vi "SetRunOptions.vi"(7 "Options":T1={"exclude instances?"=FALSE, "exclude external? (T)"=TRUE, "separate tests?"=FALSE, "top level results only?"=FALSE, "Export options"={"Export rules"=FALSE, "Export dependencies"=FALSE, "Export invalid dependencies"=FALSE, "Export concessions"=FALSE, "Export undeclared"=FALSE}, "Filter options"={"Source filter"=refnum, "Target filter"=refnum, "AND Condition?"=FALSE}}, 8 "error in (no error)":errorcluster, 10 "Root path":path, 11 "CDependencyInspection in":refnum<class "CDependencyInspection.lvclass">) -> (0 "error out":errorcluster, 3 "CDependencyInspection out":refnum<class "CDependencyInspection.lvclass">)   [LabVIEW 2020, in "DependencyInspection.lvlib" / "CDependencyInspection.lvclass"]
uses:
  CDependencyInspection.lvclass
  Options.ctl
  Options_Export.ctl
  Options_Filter.ctl
  CDependencyInspection.lvclass/CDependencyInspection.ctl
  CItemMatch/CItemMatch.lvclass
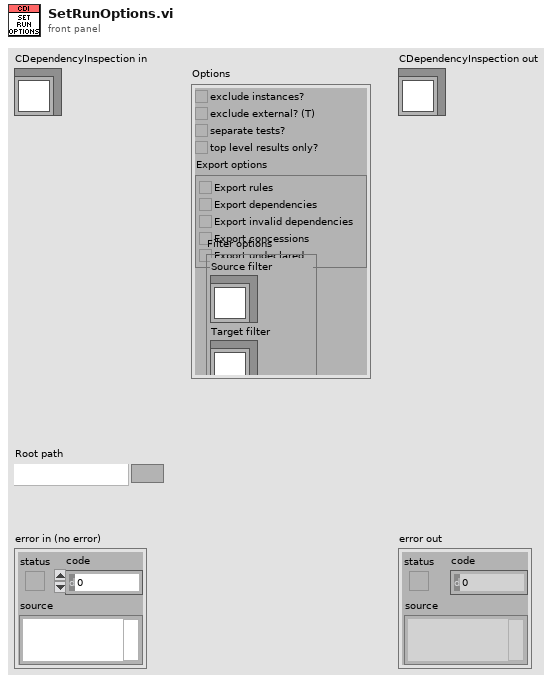
[diagram p1: front panel]
types:
  T1 = typedef "DependencyInspection.lvlib/CDependencyInspection.lvclass/Options.ctl" = cluster{"exclude instances?":bool, "exclude external? (T)":bool, "separate tests?":bool, "top level results only?":bool, "Export options":T2, "Filter options":T3}
  T2 = typedef "DependencyInspection.lvlib/CDependencyInspection.lvclass/Options_Export.ctl" = cluster{"Export rules":bool, "Export dependencies":bool, "Export invalid dependencies":bool, "Export concessions":bool, "Export undeclared":bool}
  T3 = typedef "DependencyInspection.lvlib/CDependencyInspection.lvclass/Options_Filter.ctl" = cluster{"Source filter":refnum<class "CItemMatch.lvclass">, "Target filter":refnum<class "CItemMatch.lvclass">, "AND Condition?":bool}
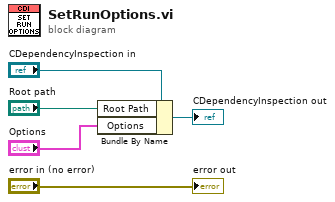
[diagram p0: block diagram]
diagram:
  n1 = Bundle By Name(cluster="CDependencyInspection in", "Root Path"="Root path", "Options"="Options") -> (→"CDependencyInspection out":refnum<class "CDependencyInspection.lvclass">)
  "error out" <- "error in (no error)"
